vi "SampleDependentVI.vi"(8 "error in (no error)":errorcluster, 11 "SampleDependentClass in":refnum<class "SampleDependentClass.lvclass">) -> (0 "error out":errorcluster, 3 "SampleDependentClass out":refnum<class "SampleDependentClass.lvclass">)   [LabVIEW 2019, in "SampleDependentLib.lvlib" / "SampleDependentClass.lvclass"]
uses:
  SampleDependentClass.lvclass
  <vilib>/xml/Load XML File.vi
  <vilib>/xml/NI_XML.lvlib
  ExternalDep/ExternalDepClass/ExternalDepClass.lvclass
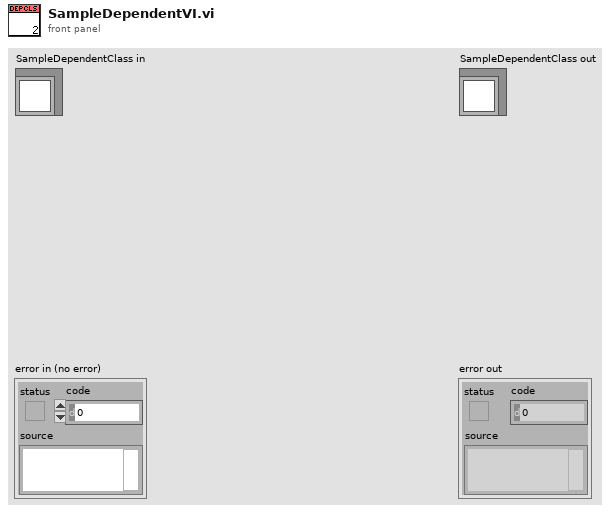
[diagram p1: front panel]
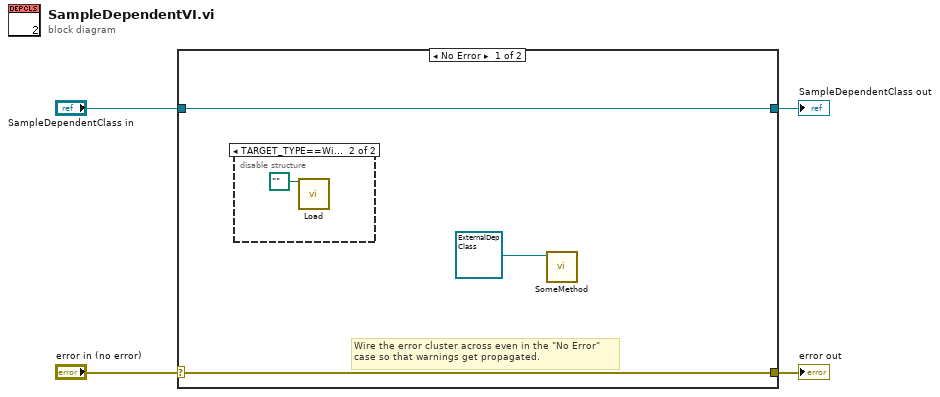
[diagram p0: block diagram]
diagram:
  n1 = case shown="No Error" "error in (no error)" {
    selector: "error in (no error)" -> [w6 w10]
    tunnel: [w6 w10] -> w3
    tunnel: [w7 w9] -> w1
    tunnel: "SampleDependentClass in" -> [w7 w9]
    frame No Error {
      # "Wire the error cluster across even in the \"No Error\"\ncase so that warnings get propagated."
      n2 = disable-structure shown="TARGET_TYPE==Windows" {
        frame condition #0 {
        }
        frame condition #1 (active) {
          n3 = call-poly <vilib>:"Load.vi"("path to XML document"=path "") -> ()  [unwired: 12 in, 3 out]
        }
      }
      n4 = call-dynamic "SomeMethod.vi"("ExternalDepClass in"=refnum<class "ExternalDepClass.lvclass"> refnum ("ExternalDep.lvlib:ExternalDepClass.lvclass")) -> ()  [unwired: 9 in, 2 out]
    }
    frame Error {
    }
  }
  "error out" <- w3
  "SampleDependentClass out" <- w1
